vi "Cache Panel Blank.vi"(8 "error in (no error)":errorcluster, 11 "2DArrayManager in":refnum<class "2DArrayManager.lvclass">) -> (0 "error out":errorcluster, 3 "2DArrayManager out":refnum<class "2DArrayManager.lvclass">)   [LabVIEW 2020, in "OOPanel.lvlib" / "2DArrayManager.lvclass"]
uses:
  2DArrayManager.lvclass
  2DArrayManager.lvclass/2DArrayManager.ctl
  2DPanelBlank/2DPanelBlank.lvclass
  C:/dev/lv20CE/relink/lv-oopanel/OOPanel/Panel/Panel.lvclass
  Manager/Manager.lvclass
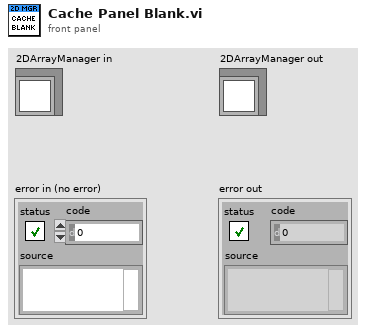
[diagram p1: front panel]
types:
  T1 = typedef "OOPanel.lvlib/2DArrayManager.lvclass/Options.ctl" = cluster{"Running":bool, "Borders":bool, "Background":u32, "V Scroll":bool, "H Scroll":bool, "Blank":refnum<class "2DPanelBlank.lvclass">, "Initial Blank Count":i32}
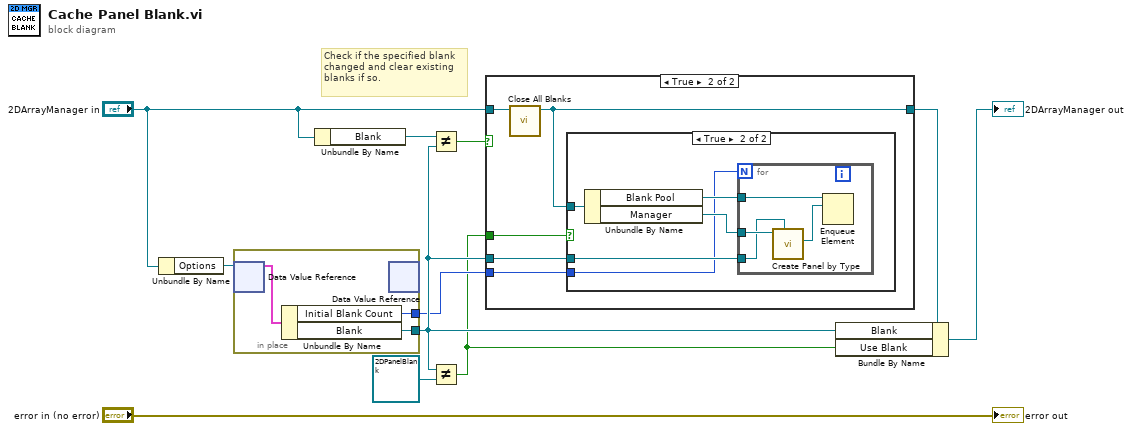
[diagram p0: block diagram]
diagram:
  # "Check if the specified blank changed and clear existing blanks if so."
  n1 = Unbundle By Name("2DArrayManager in") -> ("Options"=w10:refnum<data-value>)
  n2 = in-place {
    in-place-border: [w13] -> w4
    in-place-border: [w12] -> w3
    n3 = in-place-dvr #1(w10) -> (w14:T1)  [unwired: 1 out]
    n4 = Unbundle By Name(w14) -> ("Initial Blank Count"=w12:i32, "Blank"=w13:refnum<class "2DPanelBlank.lvclass">)
    n5 = in-place-dvr #1() -> ()  [unwired: 1 in, 2 out]
  }
  n6 = Unbundle By Name("2DArrayManager in") -> ("Blank"=w8:refnum<class "2DPanelBlank.lvclass">)
  n7 = Not Equal?(x=w8, y=w4) -> (x != y?=w5:bool)
  n8 = Not Equal?(x=w4, y=refnum<class "2DPanelBlank.lvclass"> refnum) -> (x != y?=w2:bool)
  n9 = case shown="True" w5 {
    tunnel: "2DArrayManager in" -> [w15 w20]
    tunnel: [w15 w19] -> w7
    tunnel: w4 -> [_ w18]
    tunnel: w3 -> [_ w17]
    tunnel: w2 -> [_ w16]
    frame False {
    }
    frame True {
      n10 = call "Close All Blanks.vi"("2DArrayManager in"=w20) -> ("2DArrayManager out"=w19:refnum<class "2DArrayManager.lvclass">)  [unwired: 9 in, 1 out]
      n11 = case shown="True" w16 {
        tunnel: w19 -> [_ w25]
        tunnel: w18 -> [_ w23]
        tunnel: w17 -> [_ w21]
        frame False {
        }
        frame True {
          n12 = Unbundle By Name(w25) -> ("Blank Pool"=w22:refnum<queue>, "Manager"=w24:refnum<class "Manager.lvclass">)
          n13 = for {
            N: w21 -> [_]
            tunnel: w24 -> [w29]
            tunnel: w23 -> [w28]
            tunnel: w22 -> [w27]
            n14 = call "Create Panel by Type.vi"("Panel Type"=w28, "Manager in"=w29) -> ("Panel"=w26:refnum<class "2DPanelBlank.lvclass">)  [unwired: 7 in, 2 out]
            n15 = Enqueue Element(queue=w27, element=w26) -> ()  [unwired: 2 in, 3 out]
          }
        }
      }
    }
  }
  n16 = Bundle By Name(cluster=w7, "Blank"=w4, "Use Blank"=w2) -> (→"2DArrayManager out":refnum<class "2DArrayManager.lvclass">)
  "error out" <- "error in (no error)"
